vi "get_roll_serial_test.vi"() -> ()   [LabVIEW 2026]
panel:
  out "from ESP32?":bool
  out "roll":i32
  in  "ESP32_Data":refnum<visa-resource-name>="COM20"
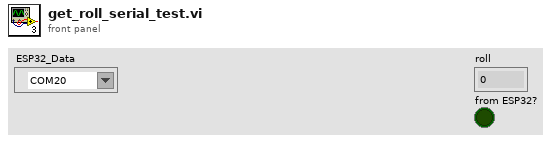
[diagram p1: front panel]
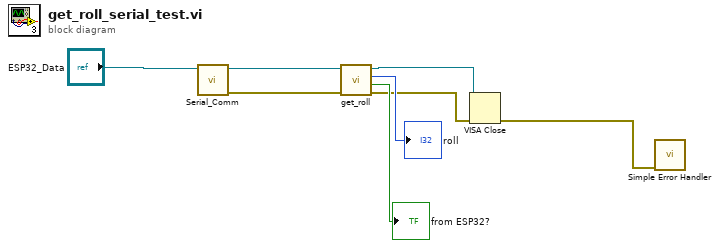
[diagram p0: block diagram]
diagram:
  n1 = call "Serial_Comm.vi"("ESP32_Data"="ESP32_Data") -> ("Roll_result"=w7:refnum<visa-resource-name>, "error out"=w3:errorcluster)  [unwired: 8 in]
  n2 = call "get_roll.vi"("error in (no error)"=w3, "ESP32 TRNG"=w7) -> ("error out"=w2:errorcluster, "from ESP32?"=→"from ESP32?":bool, "roll"=→"roll":i32, "ESP32 TRNG"=w6:refnum<visa-resource-name>)  [unwired: 6 in]
  n3 = VISA Close(VISA resource name=w6, error in (no error)=w2) -> (error out=w1:errorcluster)
  n4 = call <vilib>:"Simple Error Handler.vi"("error in (no error)"=w1) -> ()  [unwired: 4 in, 5 out]
